vi "Add Type Specifier Constant to Frame.vi"(8 "error in (no error)":errorcluster, 10 "Frame In":refnum<vi>, 11 "Setter Generator In":refnum<class "Setter Generator.lvclass">) -> (0 "error out":errorcluster, 2 "Frame Out":refnum<vi>, 3 "Setter Generator Out":refnum<class "Setter Generator.lvclass">)   [LabVIEW 2020, in "Method Generation.lvlib" / "Setter Generator.lvclass"]
uses:
  Setter Generator.lvclass
  <vilib>/Utility/miscctls.llb/LVPointTypeDef.ctl
  Setter Generator.lvclass/Setter Generator.ctl
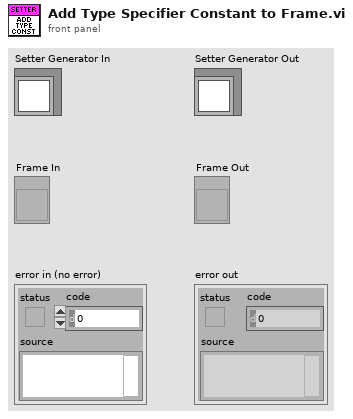
[diagram p1: front panel]
types:
  T1 = typedef "LVPointTypeDef.ctl" = cluster{"Horizontal":i16, "Vertical":i16}
  T2 = typedef "LVBoundsTypeDef.ctl" = cluster{"Width":u32, "Height":u32}
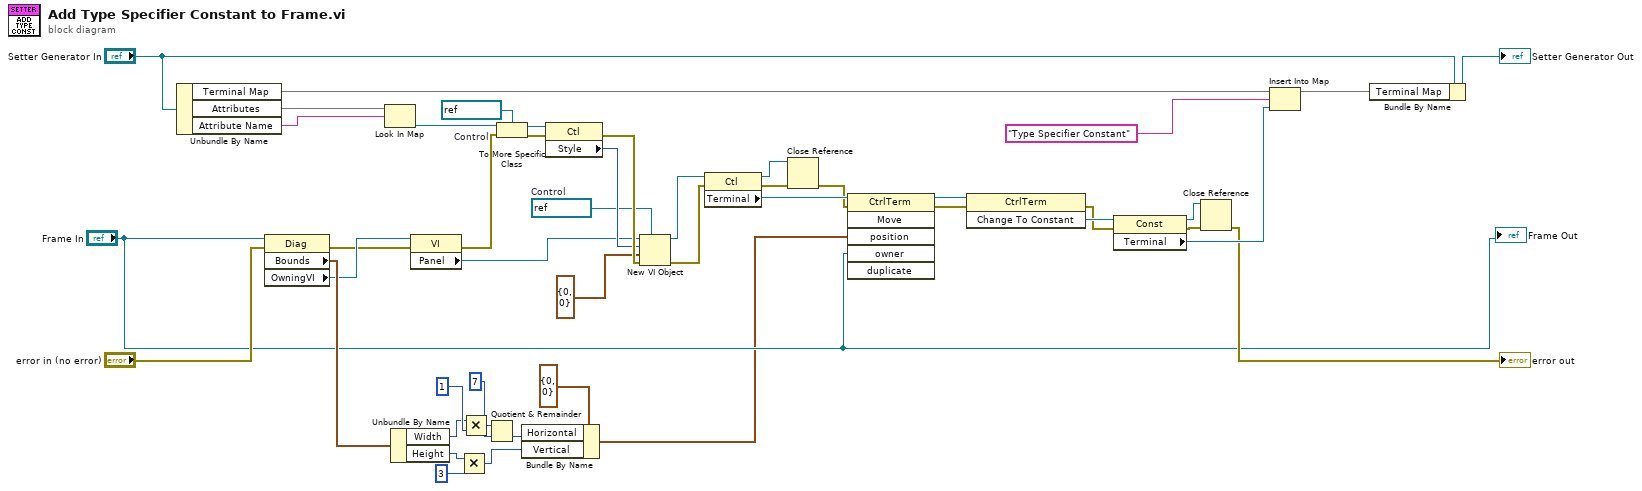
[diagram p0: block diagram]
diagram:
  w37 = refnum<vi> refnum  # Control
  w42 = refnum<vi> refnum  # Control
  n1 = Unbundle By Name("Setter Generator In") -> ("Terminal Map"=w27:map{string, refnum<vi>}, "Attributes"=w46:map{string, refnum<vi>}, "Attribute Name"=w45:string)
  n2 = property class="Diag"(reference="Frame In", error in="error in (no error)") -> (error out=w10:errorcluster, "Bounds"=w15:T2, "OwningVI"=w11:refnum<vi>)  [unwired: 1 out]
  n3 = Look In Map(map=w46, key=w45) -> (value=w40:refnum<vi>)  [unwired: 1 in, 1 out]
  n4 = Unbundle By Name(w15) -> ("Width"=w17:u32, "Height"=w23:u32)
  n5 = property class="VI"(reference=w11, error in=w10) -> (error out=w9:errorcluster, "Panel"=w8:refnum<vi>)  [unwired: 1 out]
  n6 = Multiply(x=w23, y=u32 3) -> (x*y=w21:u32)
  n7 = Multiply(x=w17, y=u32 1) -> (x*y=w19:u32)
  n8 = Quotient & Remainder(x=w19, y=u32 7) -> (floor(x/y)=w22:u32)  [unwired: 1 out]
  n9 = To More Specific Class(target class=w42, reference=w40, error in=w9) -> (specific class reference=w43:refnum<vi>, error out=w41:errorcluster)
  n10 = Bundle By Name(cluster=T1 {"Horizontal"=0, "Vertical"=0} ("location"), "Horizontal"=w22, "Vertical"=w21) -> (w5:T1)
  n11 = property class="Ctl"(reference=w43, error in=w41) -> (error out=w39:errorcluster, "Style"=w38:u32)  [unwired: 1 out]
  n12 = New VI Object(vi object class=w37, owner refnum=w8, style=w38, position/next to=T1 {"Horizontal"=0, "Vertical"=0} ("location"), 8:w39) -> (object refnum=w30:refnum<vi>, 0:w12:errorcluster)  [unwired: 3 in]
  n13 = property class="Ctl"(reference=w30, error in=w12) -> (reference out=w32:refnum<vi>, error out=w36:errorcluster, "Terminal"=w4:refnum<vi>)
  n14 = Close Reference(reference=w32, error in (no error)=w36) -> (error out=w2:errorcluster)
  n15 = invoke class="CtrlTerm" method="Move"(reference=w4, error in=w2, "position"=w5, "owner"="Frame In") -> (reference out=w3:refnum<vi>, error out=w1:errorcluster)  [unwired: 2 in, 4 out]
  n16 = invoke class="CtrlTerm" method="Change To Constant"(reference=w3, error in=w1) -> (error out=w34:errorcluster, "Change To Constant"=w35:refnum<vi>)  [unwired: 1 in, 1 out]
  n17 = property class="Const"(reference=w35, error in=w34) -> (reference out=w31:refnum<vi>, error out=w33:errorcluster, "Terminal"=w25:refnum<vi>)
  n18 = Close Reference(reference=w31, error in (no error)=w33) -> (error out=→"error out":errorcluster)
  n19 = Insert Into Map(map in=w27, key="Type Specifier Constant", value=w25) -> (map out=w28:map{string, refnum<vi>})  [unwired: 2 out]
  n20 = Bundle By Name(cluster="Setter Generator In", "Terminal Map"=w28) -> (→"Setter Generator Out":refnum<class "Setter Generator.lvclass">)
  "Frame Out" <- "Frame In"
